vi "Increment.vi"(8 "error in (no error)":errorcluster, 11 "Viewmodel in":refnum<class "Viewmodel.lvclass">) -> (0 "error out":errorcluster, 3 "Viewmodel out":refnum<class "Viewmodel.lvclass">)   [LabVIEW 2024, in "Viewmodel.lvclass"]
uses:
  Viewmodel.lvclass
  C:/Users/N Tan/Documents/1-Reuse Modules/ReactiveState/ChangeNotifier/ChangeNotifier.lvclass
  Viewmodel.lvclass/Viewmodel.ctl
  ChangeNotifier/ChangeNotifier.lvclass
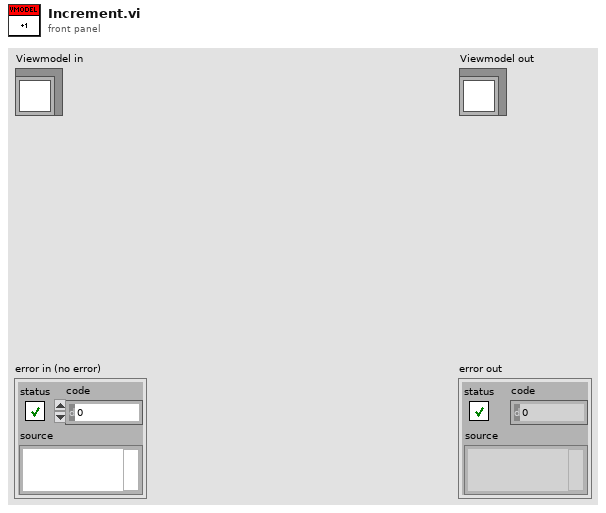
[diagram p1: front panel]
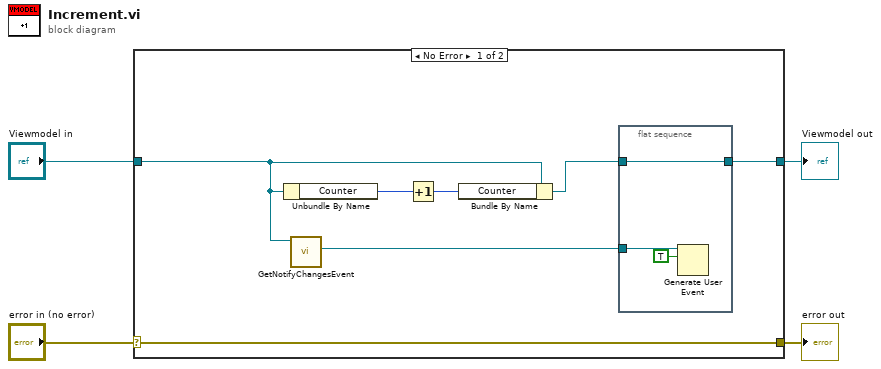
[diagram p0: block diagram]
diagram:
  n1 = case shown="No Error" "error in (no error)" {
    selector: "error in (no error)" -> [w11 w16]
    tunnel: [w11 w16] -> w3
    tunnel: [w5 w15] -> w1
    tunnel: "Viewmodel in" -> [w7 w15]
    frame No Error {
      n2 = Unbundle By Name(w7) -> ("Counter"=w8:i32)
      n3 = call "GetNotifyChangesEvent.vi"("ChangeNotifier in"=w7) -> ("notifyChangesEvent"=w9:refnum<user-event>)  [unwired: 8 in, 2 out]
      n4 = Increment(x=w8) -> (x+1=w10:i32)
      n5 = Bundle By Name(cluster=w7, "Counter"=w10) -> (w6:refnum<class "Viewmodel.lvclass">)
      n6 = flat-sequence {
        tunnel: w9 -> [w13]
        tunnel: w6 -> [w12]
        tunnel: [w12] -> w5
        frame #0 {
          n7 = Generate User Event(user event=w13, event data cluster=TRUE ("event data")) -> ()  [unwired: 2 in, 2 out]
        }
      }
    }
    frame Error {
    }
  }
  "error out" <- w3
  "Viewmodel out" <- w1
